vi "GenerateNavigationPages.vi"(2 "Root Directory":path, 3 "VI Documentation Pages":path[](array[path]), 4 "Project name":string="<Project Name>") -> ()   [LabVIEW 2019, in "ArgosLib.lvlib"]
uses:
  ArgosLib.lvlib
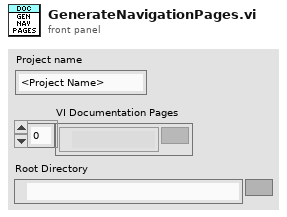
[diagram p1: front panel]
types:
  T1 = enum16{"open", "replace", "create", "open or create", "replace or create", "replace or create with confirmation"}
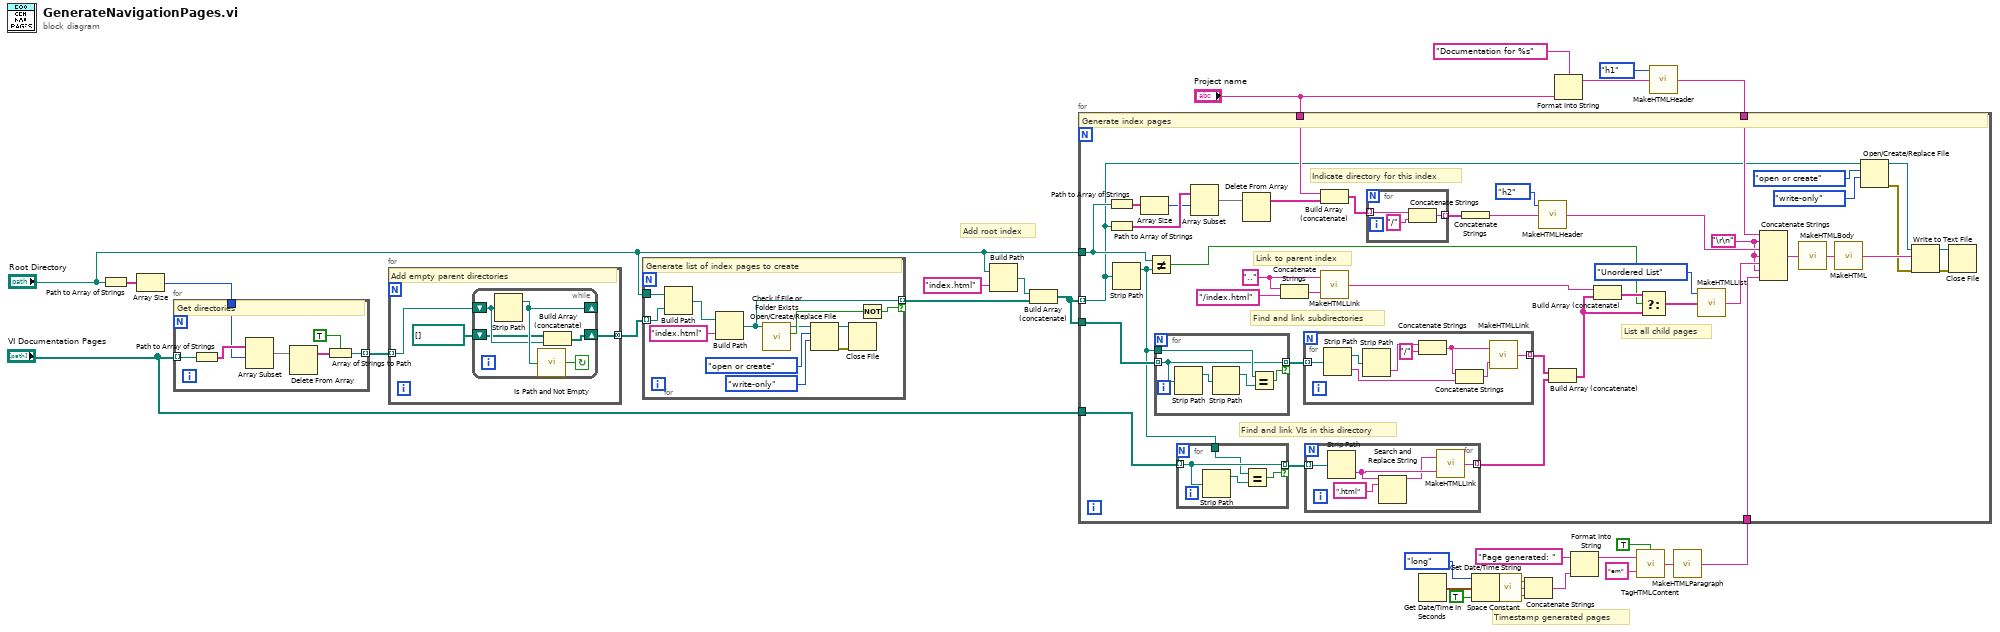
[diagram p0: block diagram]
diagram:
  # "Timestamp generated pages"
  # "Add root index"
  n1 = Path to Array of Strings(0:"Root Directory") -> (2:w28:string[])  [unwired: 1 out]
  n2 = Array Size(array=w28) -> (size(s)=w27:i32)
  n3 = for {
    tunnel: "VI Documentation Pages" -> [w35] mode=indexing
    tunnel: w27 -> [w33]
    tunnel: [w30] -> w2 mode=indexing
    # "Get directories"
    n4 = Path to Array of Strings(0:w35) -> (2:w34:string[])  [unwired: 1 out]
    n5 = Array Subset(array=w34, index=w33) -> (w32:string[])  [unwired: 1 in]
    n6 = Delete From Array(array=w32) -> (array with subset deleted=w31:string[])  [unwired: 2 in, 1 out]
    n7 = Array of Strings to Path(0:w31, 1:TRUE ("relative")) -> (2:w30:path)
  }
  n8 = for {
    tunnel: w2 -> [w38] mode=indexing
    tunnel: [w37] -> w1 mode=concatenating
    # "Add empty parent directories"
    n9 = while {
      shift-right: [w42] -> _
      shift-left: w38 -> [w41]
      shift-right: [w40] -> w37
      shift-left: path[] [] -> [w39]
      stop <- w43 continue-if-true
      n10 = Strip Path(path=w41) -> (stripped path=w42:path)  [unwired: 1 out]
      n11 = call <vilib>:"Is Path and Not Empty.vi"("path"=w42) -> ("Is Path and Not Empty?"=w43:bool)  [unwired: 4 in]
      n12 = Build Array (concatenate)(w39, w41) -> (w40:path[])
    }
  }
  n13 = for {
    tunnel: w1 -> [w55] mode=indexing
    tunnel: "Root Directory" -> [w54]
    tunnel: [w51] -> w7 mode=indexing if=w50
    # "Generate list of index pages to create"
    n14 = Build Path(base path=w54, name or relative path=w55) -> (appended path=w53:path)
    n15 = Build Path(base path=w53, name or relative path="index.html") -> (appended path=w51:path)
    n16 = call <vilib>:"Check if File or Folder Exists.vi"("path"=w51) -> ("file or folder exists?"=w49:bool, "dup path"=w48:path)  [unwired: 8 in, 1 out]
    n17 = Open/Create/Replace File(file path (use dialog)=w48, operation (0:open)=T1."open or create", access (0:read/write)=enum16{"read/write", "read-only", "write-only"}."write-only") -> (refnum out=w44:refnum<file>, error out=w45:errorcluster)  [unwired: 3 in, 1 out]
    n18 = Close File(refnum=w44, error in=w45) -> ()  [unwired: 2 out]
    n19 = Not(x=w49) -> (.not. x?=w50:bool)
  }
  n20 = Build Path(base path="Root Directory", name or relative path="index.html") -> (appended path=w5:path)
  n21 = Build Array (concatenate)(w5, w7) -> (w6:path[])
  n22 = Get Date/Time In Seconds() -> (seconds since 1Jan1904=w22:timestamp)
  n23 = Get Date/Time String(date format (0)=enum16{"short", "long", "abbreviated"}."long", seconds (now)=w22, want seconds? (F)=TRUE) -> (date string=w21:string, time string=w20:string)
  n24 = call <vilib>:"Space Constant.vi"() -> ("String"=w19:string)
  n25 = Concatenate Strings(w21, w19, w20) -> (w17:string)
  n26 = Format Into String(format string="Documentation for %s", "Project name") -> (resulting string=w24:string)  [unwired: 2 in, 1 out]
  n27 = Format Into String(initial string="Page generated: ", w17) -> (resulting string=w14:string)  [unwired: 2 in, 1 out]
  n28 = call "TagHTMLContent.vi"("Escape Contents"=TRUE, "Tag"="em", "Element Contents"=w14) -> ("Tagged Contents"=w12:string)
  n29 = call "MakeHTMLHeader.vi"("Header Content"=w24, "Header Type"=enum16{"h1", "h2", "h3", "h4", "h5", "h6"}."h1") -> ("Header Element"=w11:string)  [unwired: 3 in]
  n30 = call "MakeHTMLParagraph.vi"("Paragraph Content"=w12) -> ("Paragraph Element"=w10:string)  [unwired: 4 in]
  n31 = for {
    tunnel: w11 -> [w69]
    tunnel: w10 -> [w80]
    tunnel: w6 -> [w65] mode=indexing
    tunnel: w6 -> [w96]
    tunnel: "VI Documentation Pages" -> [w97]
    tunnel: "Root Directory" -> [w79]
    tunnel: "Project name" -> [w75]
    w68 = "\r\n"
    w88 = ".." ("string")
    # "Indicate directory for this index"
    # "Link to parent index"
    # "Find and link subdirectories"
    # "Find and link VIs in this directory"
    # "List all child pages"
    # "Generate index pages"
    n32 = Path to Array of Strings(0:w79) -> (2:w78:string[])  [unwired: 1 out]
    n33 = Path to Array of Strings(0:w65) -> (2:w77:string[])  [unwired: 1 out]
    n34 = Strip Path(path=w65) -> (stripped path=w95:path)  [unwired: 1 out]
    n35 = Array Size(array=w78) -> (size(s)=w76:i32)
    n36 = Not Equal?(x=w79, y=w95) -> (x != y?=w84:bool)
    n37 = for {
      tunnel: w96 -> [w115] mode=indexing
      tunnel: w95 -> [w116]
      tunnel: [w115] -> w94 mode=indexing if=w114
      n38 = Strip Path(path=w115) -> (stripped path=w118:path)  [unwired: 1 out]
      n39 = Strip Path(path=w118) -> (stripped path=w117:path)  [unwired: 1 out]
      n40 = Equal?(x=w116, y=w117) -> (x = y?=w114:bool)
    }
    n41 = for {
      tunnel: w97 -> [w122] mode=indexing
      tunnel: w95 -> [w120]
      tunnel: [w122] -> w93 mode=indexing if=w119
      n42 = Strip Path(path=w122) -> (stripped path=w121:path)  [unwired: 1 out]
      n43 = Equal?(x=w120, y=w121) -> (x = y?=w119:bool)
    }
    n44 = Array Subset(array=w77, index=w76) -> (w57:string[])  [unwired: 1 in]
    n45 = Delete From Array(array=w57) -> (array with subset deleted=w56:string[])  [unwired: 2 in, 1 out]
    n46 = Concatenate Strings(w88, "/index.html" ("string")) -> (w87:string)
    n47 = for {
      tunnel: w94 -> [w113] mode=indexing
      tunnel: [w106] -> w92 mode=indexing
      n48 = Strip Path(path=w113) -> (stripped path=w112:path, name=w109:string)
      n49 = Strip Path(path=w112) -> (name=w111:string)  [unwired: 1 out]
      n50 = Concatenate Strings(w111, "/" ("string")) -> (w107:string)
      n51 = Concatenate Strings(w107, w109) -> (w108:string)
      n52 = call "MakeHTMLLink.vi"("Link Target"=w108, "Link Text"=w107) -> ("HTML Link"=w106:string)
    }
    n53 = for {
      tunnel: w93 -> [w105] mode=indexing
      tunnel: [w101] -> w91 mode=indexing
      n54 = Strip Path(path=w105) -> (name=w103:string)  [unwired: 1 out]
      n55 = Search and Replace String(input string=w103, search string=".html") -> (result string=w102:string)  [unwired: 6 in, 3 out]
      n56 = call "MakeHTMLLink.vi"("Link Target"=w103, "Link Text"=w102) -> ("HTML Link"=w101:string)
    }
    n57 = Build Array (concatenate)(w75, w56) -> (w74:string[])
    n58 = call "MakeHTMLLink.vi"("Link Target"=w87, "Link Text"=w88) -> ("HTML Link"=w86:string)
    n59 = for {
      tunnel: w74 -> [w100] mode=indexing
      tunnel: [w98] -> w73 mode=indexing
      n60 = Concatenate Strings(w100, "/" ("string")) -> (w98:string)
    }
    n61 = Concatenate Strings(w73) -> (w71:string)
    n62 = call "MakeHTMLHeader.vi"("Header Content"=w71, "Header Type"=enum16{"h1", "h2", "h3", "h4", "h5", "h6"}."h2") -> ("Header Element"=w70:string)  [unwired: 3 in]
    n63 = Build Array (concatenate)(w92, w91) -> (w83:string[])
    n64 = Build Array (concatenate)(w86, w83) -> (w85:string[])
    n65 = Select(t=w85, s=w84, f=w83) -> (s? t:f=w82:string[])
    n66 = call "MakeHTMLList.vi"("List Elements"=w82, "List Type"=enum16{"Ordered List", "Unordered List"}."Unordered List") -> ("List"=w81:string)  [unwired: 3 in]
    n67 = Concatenate Strings(w69, w68, w70, w68, w81, w68, w80) -> (w66:string)
    n68 = call "MakeHTMLBody.vi"("Body Content"=w66) -> ("Body Element"=w67:string)  [unwired: 4 in]
    n69 = call "MakeHTML.vi"("HTML Content"=w67) -> ("HTML Element"=w62:string)  [unwired: 4 in]
    n70 = Open/Create/Replace File(file path (use dialog)=w65, operation (0:open)=T1."open or create", access (0:read/write)=enum16{"read/write", "read-only", "write-only"}."write-only") -> (refnum out=w61:refnum<file>, error out=w58:errorcluster)  [unwired: 3 in, 1 out]
    n71 = Write to Text File(file (use dialog)=w61, text=w62, error in=w58) -> (refnum out=w59:refnum<file>, error out=w60:errorcluster)  [unwired: 1 in, 1 out]
    n72 = Close File(refnum=w59, error in=w60) -> ()  [unwired: 2 out]
  }
